vi "R Table data formation.vi"(6 "Region Info":T2, 7 "F ex Info":T3, 8 "HPeak Cluster":T4, 9 "STD cluster":T5, 10 "BL cluster":T6, 11 "R Table C0":T1) -> (3 "appended array":string[][](array[string]))   [LabVIEW 2018]
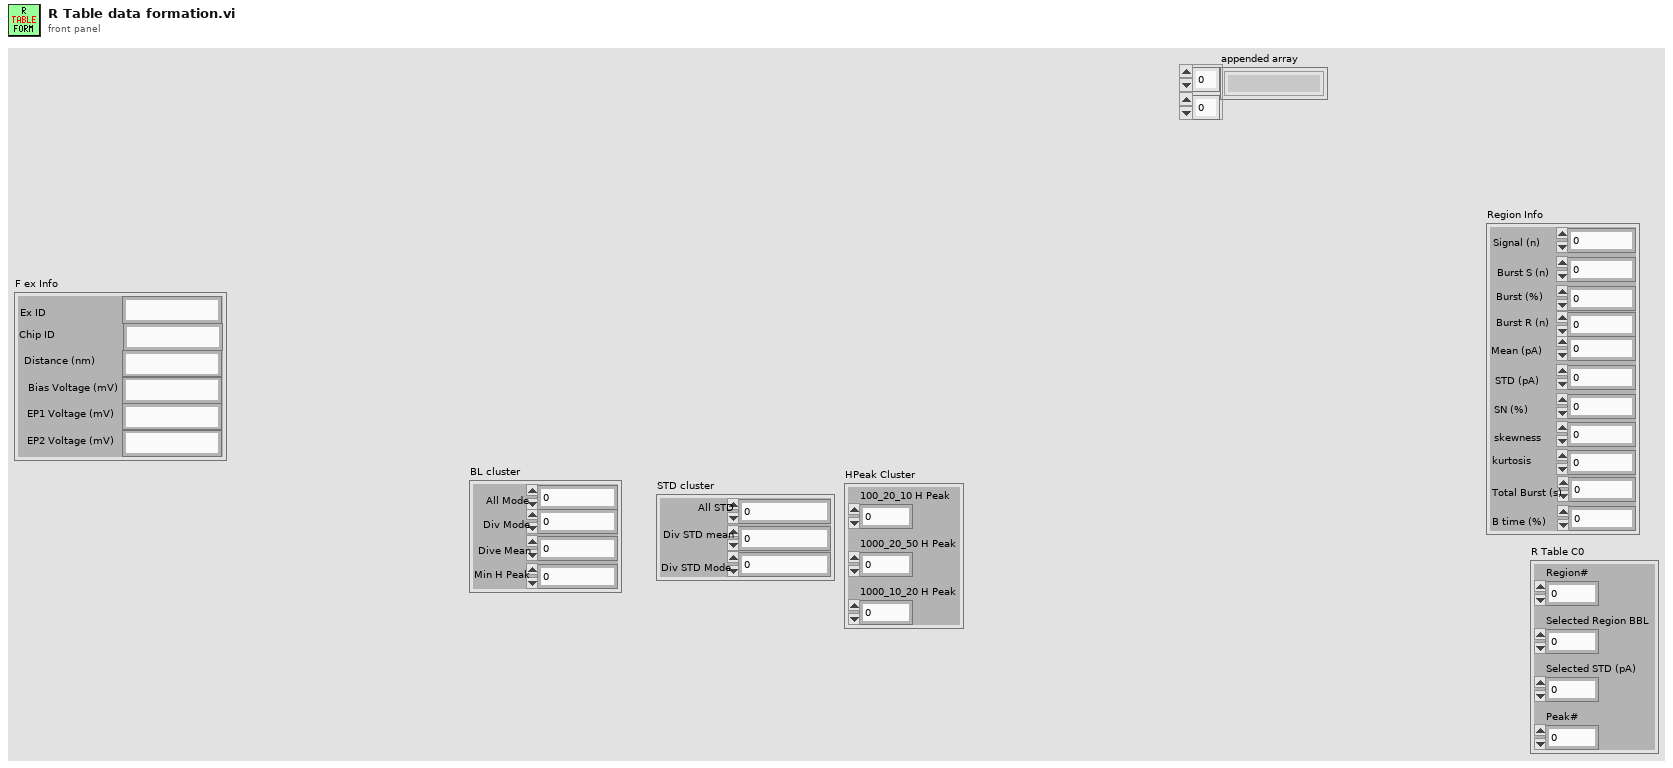
[diagram p1: front panel]
types:
  T1 = cluster{"Region#":i32, "Selected Region BBL":dbl, "Selected STD (pA)":dbl, "Peak#":i32}
  T2 = cluster{"Signal (n)":i32, "Burst S (n)":i32, "Burst (%)":dbl, "Burst R (n)":dbl, "Mean (pA)":dbl, "STD (pA)":dbl, "SN (%)":dbl, "skewness":dbl, "kurtosis":dbl, "Total Burst (s)":dbl, "B time (%)":dbl}
  T3 = cluster{"Ex ID":string, "Chip ID":string, "Distance (nm)":string, "Bias Voltage (mV)":string, "EP1 Voltage (mV)":string, "EP2 Voltage (mV)":string}
  T4 = cluster{"100_20_10 H Peak":i32, "1000_20_50 H Peak":i32, "1000_10_20 H Peak":i32}
  T5 = cluster{"All STD":dbl, "Div STD mean":dbl, "Div STD Mode":dbl}
  T6 = cluster{"All Mode":dbl, "Div Mode":dbl, "Dive Mean":dbl, "Min H Peak":dbl}
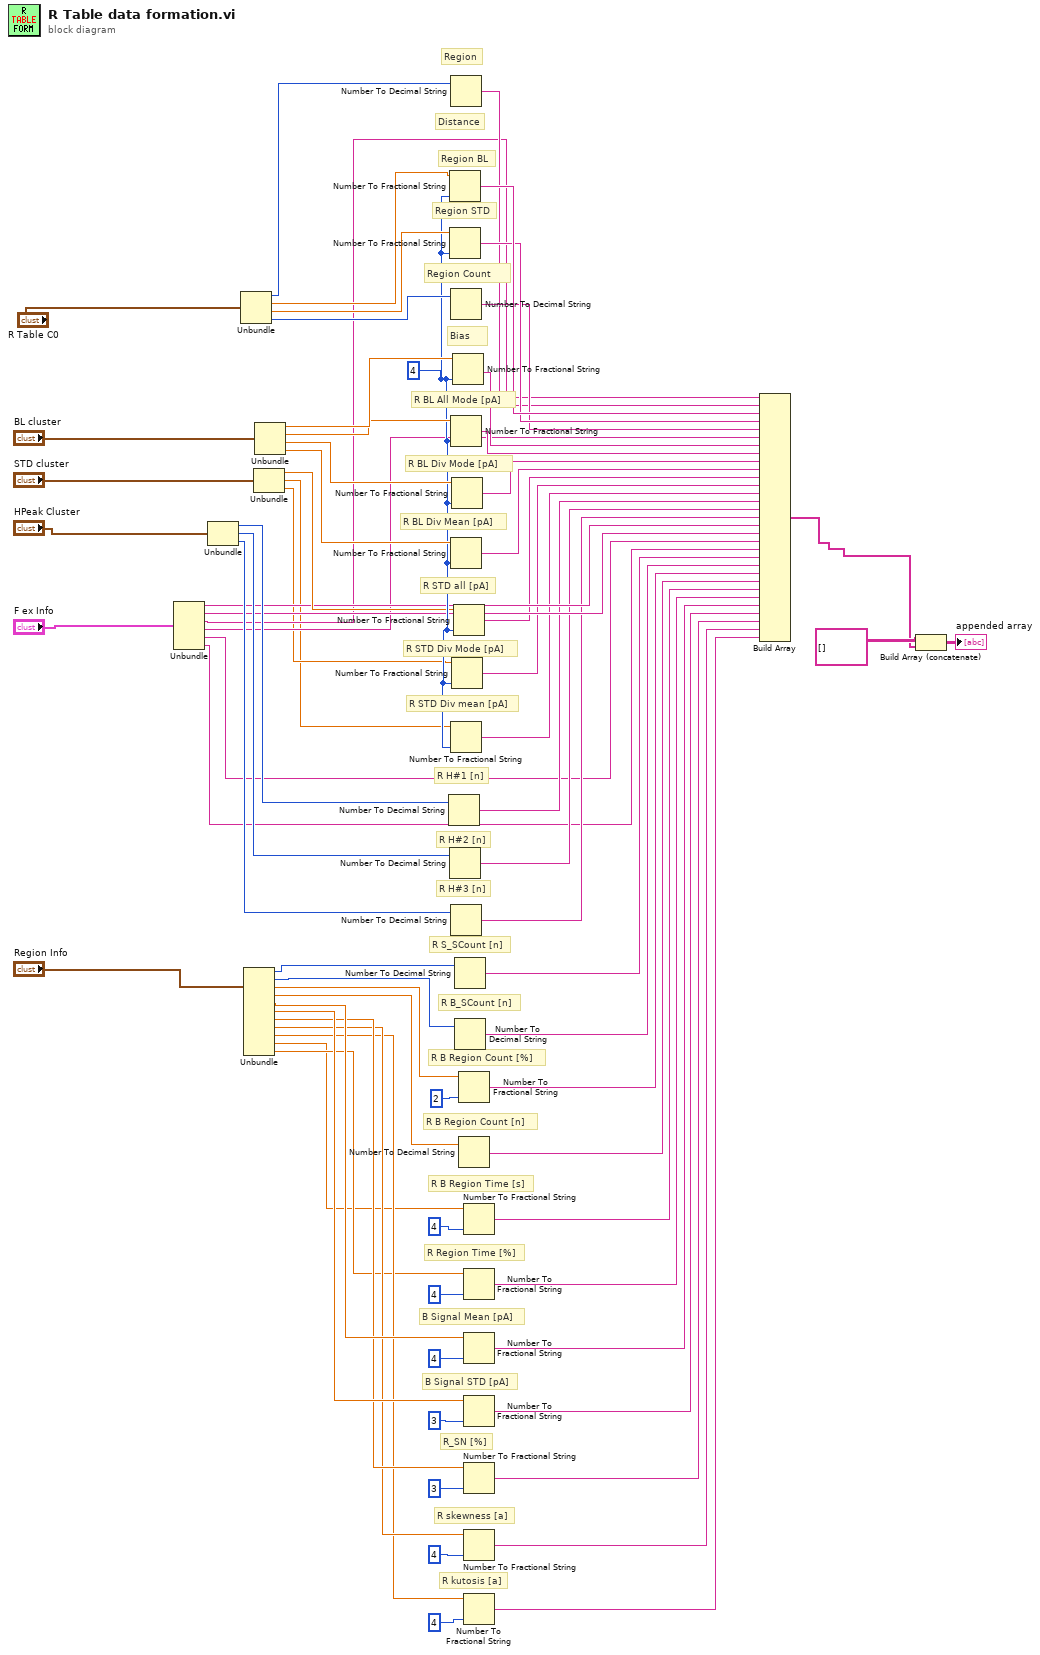
[diagram p0: block diagram]
diagram:
  w57 = i16 4 ("¸xi6j")
  # "R H#3 [n]"
  # "R H#2 [n]"
  # "R H#1 [n]"
  # "R STD Div mean [pA]"
  # "R S_SCount [n]"
  # "R B_SCount [n]"
  # "R B Region Count [%]"
  # "R B Region Count [n]"
  # "R B Region Time [s]"
  # "R Region Time [%]"
  # "B Signal Mean [pA]"
  # "B Signal STD [pA]"
  # "R_SN [%]"
  # "R skewness [a]"
  # "R kutosis [a]"
  # "R STD Div Mode [pA]"
  # "R STD all [pA]"
  # "R BL Div Mean [pA]"
  # "R BL Div Mode [pA]"
  # "R BL All Mode [pA]"
  # "Region Count"
  # "Bias"
  # "Region STD"
  # "Region BL"
  # "Region"
  # "Distance"
  n1 = Unbundle("F ex Info") -> ("Ex ID"=w51:string, "Chip ID"=w52:string, "Distance (nm)"=w41:string, "Bias Voltage (mV)"=w40:string, "EP1 Voltage (mV)"=w39:string, "EP2 Voltage (mV)"=w38:string)
  n2 = Unbundle("HPeak Cluster") -> ("100_20_10 H Peak"=w55:i32, "1000_20_50 H Peak"=w54:i32, "1000_10_20 H Peak"=w53:i32)
  n3 = Unbundle("R Table C0") -> ("Region#"=w70:i32, "Selected Region BBL"=w69:dbl, "Selected STD (pA)"=w68:dbl, "Peak#"=w67:i32)
  n4 = Unbundle("Region Info") -> ("Signal (n)"=w37:i32, "Burst S (n)"=w5:i32, "Burst (%)"=w36:dbl, "Burst R (n)"=w21:dbl, "Mean (pA)"=w29:dbl, "STD (pA)"=w28:dbl, "SN (%)"=w27:dbl, "skewness"=w26:dbl, "kurtosis"=w25:dbl, "Total Burst (s)"=w4:dbl, "B time (%)"=w16:dbl)
  n5 = Unbundle("STD cluster") -> ("All STD"=w56:dbl, "Div STD mean"=w7:dbl, "Div STD Mode"=w8:dbl)
  n6 = Unbundle("BL cluster") -> ("All Mode"=w63:dbl, "Div Mode"=w62:dbl, "Dive Mean"=w61:dbl, "Min H Peak"=w60:dbl)
  n7 = Number To Decimal String(number=w55) -> (decimal integer string=w48:string)  [unwired: 1 in]
  n8 = Number To Fractional String(number=w69, precision (6)=w57) -> (F-format string=w74:string)  [unwired: 2 in]
  n9 = Number To Fractional String(number=w68, precision (6)=w57) -> (F-format string=w73:string)  [unwired: 2 in]
  n10 = Number To Decimal String(number=w54) -> (decimal integer string=w49:string)  [unwired: 1 in]
  n11 = Number To Decimal String(number=w70) -> (decimal integer string=w71:string)  [unwired: 1 in]
  n12 = Number To Decimal String(number=w67) -> (decimal integer string=w72:string)  [unwired: 1 in]
  n13 = Number To Fractional String(number=w62, precision (6)=w57) -> (F-format string=w58:string)  [unwired: 2 in]
  n14 = Number To Fractional String(number=w60, precision (6)=w57) -> (F-format string=w44:string)  [unwired: 2 in]
  n15 = Number To Fractional String(number=w7, precision (6)=w57) -> (F-format string=w47:string)  [unwired: 2 in]
  n16 = Number To Decimal String(number=w53) -> (decimal integer string=w50:string)  [unwired: 1 in]
  n17 = Number To Fractional String(number=w61, precision (6)=w57) -> (F-format string=w43:string)  [unwired: 2 in]
  n18 = Number To Fractional String(number=w8, precision (6)=w57) -> (F-format string=w46:string)  [unwired: 2 in]
  n19 = Number To Fractional String(number=w63, precision (6)=w57) -> (F-format string=w59:string)  [unwired: 2 in]
  n20 = Number To Fractional String(number=w56, precision (6)=w57) -> (F-format string=w45:string)  [unwired: 2 in]
  n21 = Number To Decimal String(number=w37) -> (decimal integer string=w24:string)  [unwired: 1 in]
  n22 = Number To Decimal String(number=w5) -> (decimal integer string=w23:string)  [unwired: 1 in]
  n23 = Number To Fractional String(number=w36, precision (6)=i16 2 ("¸xi6j")) -> (F-format string=w22:string)  [unwired: 2 in]
  n24 = Number To Decimal String(number=w21) -> (decimal integer string=w20:string)  [unwired: 1 in]
  n25 = Number To Fractional String(number=w4, precision (6)=i16 4 ("¸xi6j")) -> (F-format string=w15:string)  [unwired: 2 in]
  n26 = Number To Fractional String(number=w16, precision (6)=i16 4 ("¸xi6j")) -> (F-format string=w14:string)  [unwired: 2 in]
  n27 = Number To Fractional String(number=w29, precision (6)=i16 4 ("¸xi6j")) -> (F-format string=w13:string)  [unwired: 2 in]
  n28 = Number To Fractional String(number=w28, precision (6)=i16 3 ("¸xi6j")) -> (F-format string=w12:string)  [unwired: 2 in]
  n29 = Number To Fractional String(number=w27, precision (6)=i16 3 ("¸xi6j")) -> (F-format string=w11:string)  [unwired: 2 in]
  n30 = Number To Fractional String(number=w26, precision (6)=i16 4 ("¸xi6j")) -> (F-format string=w10:string)  [unwired: 2 in]
  n31 = Number To Fractional String(number=w25, precision (6)=i16 4 ("¸xi6j")) -> (F-format string=w9:string)  [unwired: 2 in]
  n32 = Build Array(w71, w41, w74, w73, w72, w40, w59, w58, w43, w44, w45, w46, w47, w48, w49, w50, w51, w52, w39, w38, w24, w23, w22, w20, w15, w14, w13, w12, w11, w10, w9) -> (w2:string[])
  n33 = Build Array (concatenate)(string[][] [], w2) -> (→"appended array":string[][])
